vi "Start Acq.vi"(6 "Rec File":string, 8 "error in (no error)":errorcluster, 9 "Write to disk":bool, 10 "Frame Count":i32=-1, 11 "HamamatsuFluor in":refnum<class "HamamatsuFluor.lvclass">) -> (0 "error out":errorcluster, 2 "File path":path, 3 "HamamatsuFluor out":refnum<class "HamamatsuFluor.lvclass">)   [LabVIEW 2020, in "DAQ Timed SPIM.lvlib" / "HamamatsuFluor_v2.lvlib" / "HamamatsuFluor.lvclass"]
uses:
  HamamatsuFluor.lvclass
  D:/wcalhoun6/Dropbox (GaTech)/LabView/SPIM Engine/HW Timed SPIM/Abstract DAQ Triggered Actor/Abstract DAQ Triggered Actor.lvclass
  HamamatsuFluor.lvclass/HamamatsuFluor.ctl
  Abstract DAQ Triggered Actor/Abstract DAQ Triggered Actor.lvclass/Abstract DAQ Triggered Actor.ctl
  Abstract DAQ Triggered Actor/Read Save Path.vi
  WIN Memory Map.llb/WIN MMAP.lvlib
panel:
  in  "Max frames":i32=750000
  out "Frame Count 2":i32
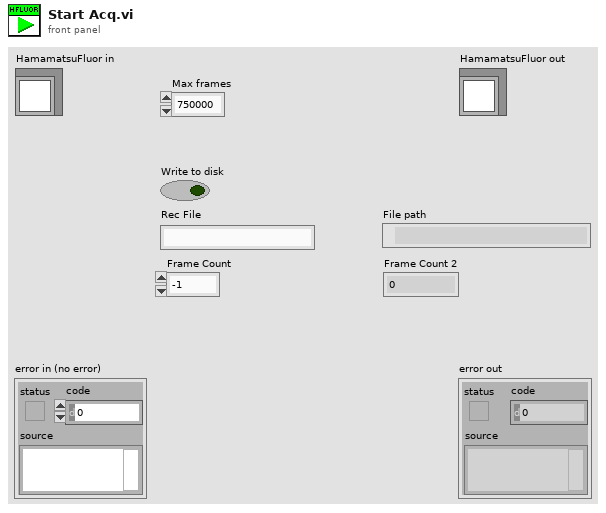
[diagram p1: front panel]
types:
  T1 = enum16{"big-endian, network order", "native, host order", "little-endian"}
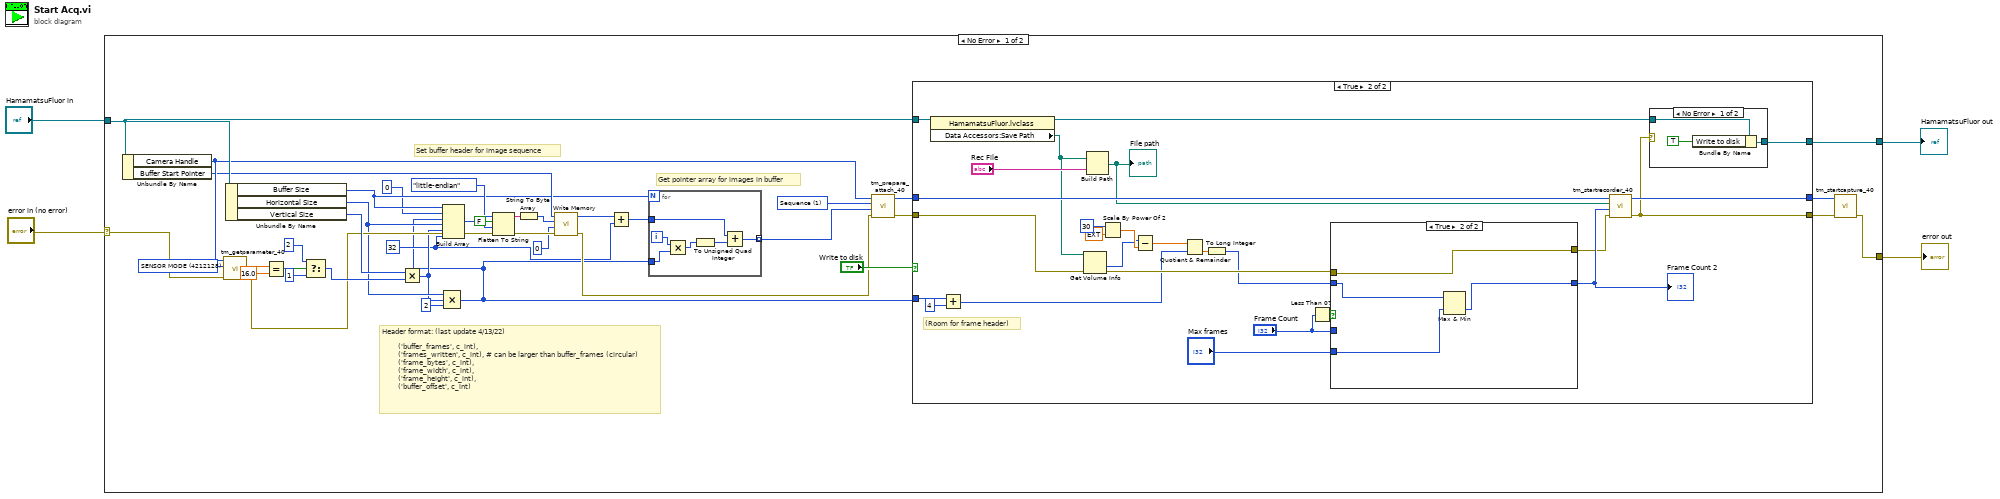
[diagram p0: block diagram]
diagram:
  n1 = case shown="No Error" "error in (no error)" {
    selector: "error in (no error)" -> [w31 w89]
    tunnel: "HamamatsuFluor in" -> [w37 w90]
    tunnel: [w40 w90] -> w1
    tunnel: [w35 w89] -> w2
    frame No Error {
      w6 = 32 ("element")
      w30 = u32 4212128 items=["SENSOR MODE"=4212128, "READOUT SPEED"=4211872, "READOUT DIRECTION"=4211904, "BIT PER CHANNEL"=4342976, "TRIGGER GLOBAL EXPOSURE"=2049680, "TRIGGER DELAY"=1066480, "INTERNAL TRIGGER HANDLING"=1066496, "SENSOR TEMPERATURE"=2115232, "SENSOR COOLER STATUS"=2115280, "EXPOSURE TIME"=2049184, "DEFECT CORRECT MODE"=4670368, "HOT PIXEL CORRECT LEVEL"=4670400, "BINNING"=4215968, "TIMING READOUT TIME"=4223904, "INTERNAL FRAME RATE"=4225952, "INTERNAL FRAME INTERVAL"=4225968, "INTERNAL LINE SPEED"=4226000, "INTERNAL LINE INTERVAL"=4226016, "IMAGE WIDTH"=4343200, "IMAGE HEIGHT"=4343216, "IMAGE ROWBYTES"=4343232, "IMAGE FRAMEBYTES"=4343248, "IMAGE PIXEL TYPE"=4343296, "NUMBER OF OUTPUT TRIGGER CONNECTOR"=1852320, "OUTPUT TRIGGER SOURCE[0]"=1852576, "OUTPUT TRIGGER SOURCE[1]"=1852832, "OUTPUT TRIGGER SOURCE[2]"=1853088, "OUTPUT TRIGGER POLARITY[0]"=1852592, "OUTPUT TRIGGER POLARITY[1]"=1852848, "OUTPUT TRIGGER POLARITY[2]"=1853104, "OUTPUT TRIGGER ACTIVE[0]"=1852608, "OUTPUT TRIGGER ACTIVE[1]"=1852864, "OUTPUT TRIGGER ACTIVE[2]"=1853120, "OUTPUT TRIGGER DELAY[0]"=1852624, "OUTPUT TRIGGER DELAY[1]"=1852880, "OUTPUT TRIGGER DELAY[2]"=1853136, "OUTPUT TRIGGER PERIOD[0]"=1852640, "OUTPUT TRIGGER PERIOD[1]"=1852896, "OUTPUT TRIGGER PERIOD[2]"=1853152, "OUTPUT TRIGGER KIND[0]"=1852656, "OUTPUT TRIGGER KIND[1]"=1852912, "OUTPUT TRIGGER KIND[2]"=1853168, "OUTPUT TRIGGER BASE SENSOR[0]"=1852672, "OUTPUT TRIGGER BASE SENSOR[1]"=1852928, "OUTPUT TRIGGER BASE SENSOR[2]"=1853184, "OUTPUT TRIGGER PRE HSYNC COUNT"=1852704] ("Parameter")
      w43 = 1 items=["Snap", "Sequence"] ("Capture mode")
      # "Header format: (last update 4/13/22)\n\n        ('buffer_frames', c_int),\n        ('frames_written', c_int), # can be larger than buffer_frames (circular)\n        ('frame_bytes', c_int),\n        ('frame_width', c_int),\n        ('frame_height', c_int),\n        ('buffer_offset', c_int)"
      # "Set buffer header for image sequence"
      # "Get pointer array for images in buffer"
      n2 = Unbundle By Name(w37) -> ("Camera Handle"=w32:u32, "Buffer Start Pointer"=w18:u64)
      n3 = call <userlib>:"tm_getparameter_40.vi"("error in (no error)"=w31, "Parameter"=w30, "Handle in"=w32) -> ("error out"=w20:errorcluster, "Value out"=w29:dbl)  [unwired: 6 in, 1 out]
      n4 = Unbundle By Name(w37) -> ("Buffer Size"=w14:i32, "Horizontal Size"=w8:i32, "Vertical Size"=w36:i32)
      n5 = Equal?(x=w29, y=16.0) -> (x = y?=w27:bool)
      n6 = Select(t=2 ("y"), s=w27, f=1) -> (s? t:f=w24:i32)
      n7 = Multiply(x=w36, y=w24) -> (x*y=w7:i32)
      n8 = Compound Arithmetic op=MULTIPLY(w8, w7, 2 ("value")) -> (w5:i32)
      n9 = Build Array(w14, 0 ("element"), w5, w8, w7, w6) -> (w23:i32[])
      n10 = Flatten To String(anything=w23, prepend array or string size? (T)=FALSE, byte order (0:big-endian, network order)=T1."little-endian", error in (no error)=w20) -> (data string=w19:string, error out=w16:errorcluster)  [unwired: 1 out]
      n11 = String To Byte Array(string=w19) -> (unsigned byte array=w17:u8[])
      n12 = call "Write Memory.vi"("error in (no error)"=w16, "offset"=u32 0, "data"=w17, "startAddress"=w18) -> ("error out"=w11:errorcluster, "startAddress out"=w13:u64)  [unwired: 6 in]
      n13 = Add(x=w13, y=w6) -> (x+y=w10:u64)
      n14 = for {
        N: w14 -> [_]
        tunnel: w5 -> [w47]
        tunnel: [w49] -> w12 mode=indexing
        tunnel: w10 -> [w46]
        i -> [w48]
        n15 = Multiply(x=w48, y=w47) -> (x*y=w45:i32)
        n16 = To Unsigned Quad Integer(1:w45) -> (0:w44:u64)
        n17 = Add(x=w46, y=w44) -> (x+y=w49:u64)
      }
      n18 = call <userlib>:"tm_prepare_attach_40.vi"("error in (no error)"=w11, "buffers"=w12, "Capture mode"=w43, "Handle in"=w32) -> ("error out"=w42:errorcluster, "Handle out"=w41:u32)  [unwired: 6 in]
      n19 = case shown="True" "Write to disk" {
        tunnel: w41 -> [w52 w78]
        tunnel: w42 -> [w51 w65]
        tunnel: [w51 w76] -> w38
        tunnel: [w52 w77] -> w39
        tunnel: w37 -> [w50 w68]
        tunnel: [w50 w75] -> w40
        tunnel: w5 -> [_ w56]
        frame False {
        }
        frame True {
          # "(Room for frame header)"
          n20 = property class="HamamatsuFluor.lvclass"(reference=w68) -> (reference out=w67:refnum<class "HamamatsuFluor.lvclass">, "Data Accessors:Save Path"=w66:path)  [unwired: 1 in, 1 out]
          n21 = Add(x=w56, y=4) -> (x+y=w54:i32)
          n22 = Get Volume Info(8:w65, 11:w66) -> (0:w64:errorcluster, 1:w60:i64)  [unwired: 4 out]
          n23 = Build Path(base path=w66, name or relative path="Rec File") -> (appended path=w69:path)
          "File path" <- w69
          n24 = Scale By Power Of 2(n=i16 30, x=ext 100.0) -> (x*2^n=w61:ext)
          n25 = Subtract(x=w60, y=w61) -> (x-y=w59:ext)
          n26 = Quotient & Remainder(x=w59, y=w54) -> (floor(x/y)=w58:ext)  [unwired: 1 out]
          n27 = To Long Integer(number=w58) -> (32bit integer=w57:i32)
          n28 = Less Than 0?(x="Frame Count") -> (x < 0?=w74:bool)
          n29 = case shown="True" w74 {
            tunnel: w64 -> [w80 w84]
            tunnel: [w79 w82] -> w73
            tunnel: [w80 w84] -> w72
            tunnel: "Frame Count" -> [w79 _]
            tunnel: w57 -> [_ w83]
            tunnel: "Max frames" -> [_ w81]
            frame False {
            }
            frame True {
              n30 = Max & Min(x=w83, y=w81) -> (min(x,y)=w82:i32)  [unwired: 1 out]
            }
          }
          "Frame Count 2" <- w73
          n31 = call <userlib>:"tm_startrecorder_40.vi"("error in (no error)"=w72, "frames"=w73, "File"=w69, "Handle in"=w78) -> ("error out"=w76:errorcluster, "Handle out"=w77:u32)  [unwired: 6 in]
          n32 = case shown="No Error" w76 {
            tunnel: w67 -> [w87 w88]
            tunnel: [w85 w88] -> w75
            frame No Error {
              n33 = Bundle By Name(cluster=w87, "Write to disk"=TRUE ("Recording")) -> (w85:refnum<class "HamamatsuFluor.lvclass">)
            }
            frame Error {
            }
          }
        }
      }
      n34 = call <userlib>:"tm_startcapture_40.vi"("error in (no error)"=w38, "Handle in"=w39) -> ("error out"=w35:errorcluster)  [unwired: 8 in, 1 out]
    }
    frame Error {
    }
  }
  "error out" <- w2
  "HamamatsuFluor out" <- w1
